vi "Load DAC Configuration.vi"(8 "error in":errorcluster, 10 "Config File refnum in":T1, 11 "DAC HMP4040 in":refnum<class "DAC HMP4040.lvclass">) -> (0 "error out":errorcluster, 2 "Config File refnum out":T1, 3 "DAC HMP4040 out":refnum<class "DAC HMP4040.lvclass">)   [LabVIEW 2019, in "DAC.lvlib" / "DAC HMP4040.lvclass"]
uses:
  DAC HMP4040.lvclass
  C:/Users/krio/Documents/LV_Projects/test-stand/App/DAC/DAC.lvclass
  <vilib>/Utility/config.llb/Config Data RefNum.ctl
  DAC.lvclass/DAC.ctl
  DAC HMP4040.lvclass/DAC HMP4040.ctl
  <vilib>/Utility/config.llb/Read Key (String).vi
  DAC.lvclass
  <vilib>/Utility/config.llb/NI_LVConfig.lvlib
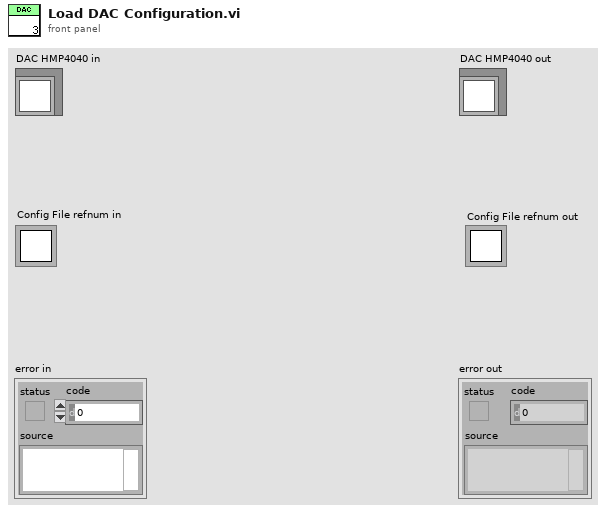
[diagram p1: front panel]
types:
  T1 = typedef "NI_LVConfig.lvlib/Config Data RefNum.ctl" = refnum<k1>
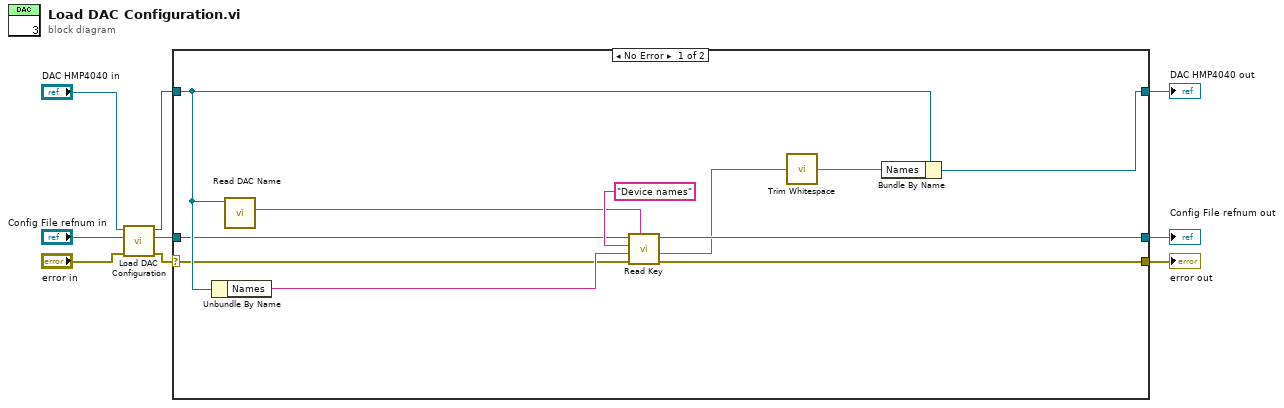
[diagram p0: block diagram]
diagram:
  n1 = call-parent "Load DAC Configuration.vi"("error in"="error in", "Config File refnum in"="Config File refnum in", "DAC in"="DAC HMP4040 in") -> ("error out"=w4:errorcluster, "Config File refnum out"=w5:T1, "DAC out"=w6:refnum<class "DAC HMP4040.lvclass">)  [unwired: 6 in]
  n2 = case shown="No Error" w4 {
    selector: w4 -> [w13 w21]
    tunnel: [w12 w23] -> w3
    tunnel: w6 -> [w19 w23]
    tunnel: w5 -> [w14 w22]
    tunnel: [w16 w22] -> w2
    tunnel: [w17 w21] -> w1
    frame No Error {
      n3 = Unbundle By Name(w19) -> ("Names"=w18:string)
      n4 = call "Read DAC Name.vi"("DAC in"=w19) -> ("DAC Name"=w15:string)  [unwired: 8 in, 2 out]
      n5 = call-poly <vilib>:"Read Key.vi"("section"=w15, "error in (no error)"=w13, "default value"=w18, "key"="Device names", "refnum"=w14) -> ("error out"=w17:errorcluster, "value"=w10:string, "refnum out"=w16:T1)  [unwired: 3 in, 1 out]
      n6 = call <vilib>:"Trim Whitespace.vi"("string"=w10) -> ("trimmed string"=w11:string)  [unwired: 1 in]
      n7 = Bundle By Name(cluster=w19, "Names"=w11) -> (w12:refnum<class "DAC HMP4040.lvclass">)
    }
    frame Error {
    }
  }
  "error out" <- w1
  "DAC HMP4040 out" <- w3
  "Config File refnum out" <- w2
